vi "Daily_Pass_Fail_Count.vi"(0 "Action":enum16{"READ", "WRITE"}(ring), 5 "Result":bool, 11 "error in":errorcluster) -> (3 "TOTAL":string, 4 "PASS":u32, 6 "FAIL":u32, 8 "PASS":string, 10 "FAIL":string, 15 "error out":errorcluster)   [LabVIEW 2021]
uses:
  controls/INI_Daily_Count_State.ctl
  <vilib>/Utility/config.llb/Write Key (I32).vi
  <vilib>/Utility/config.llb/Write Key (String).vi
  <vilib>/Utility/config.llb/Read Key (String).vi
  <vilib>/Utility/config.llb/Read Key (U32).vi
  <vilib>/Utility/config.llb/Write Key (U32).vi
  <vilib>/Utility/config.llb/NI_LVConfig.lvlib
panel:
  out "appended path":path
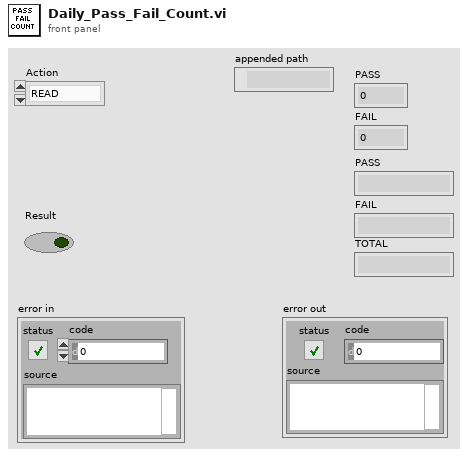
[diagram p1: front panel]
types:
  T1 = typedef "INI_Daily_Count_State.ctl" = enum16{"Check File", "Create INI File", "Check Date", "Read", "Write"}
  T2 = typedef "NI_LVConfig.lvlib/Config Data RefNum.ctl" = refnum<k1>
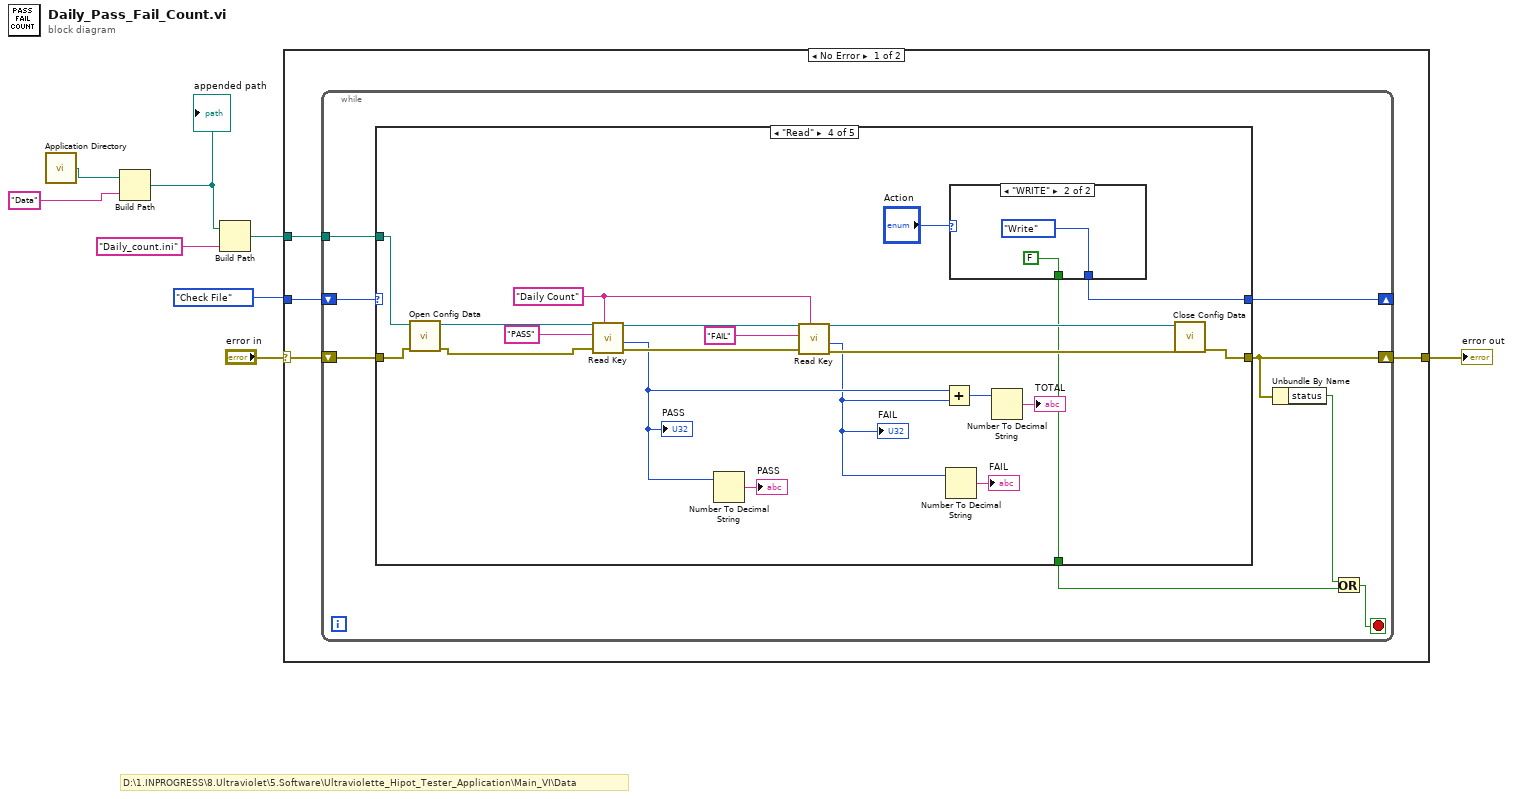
[diagram p0: block diagram]
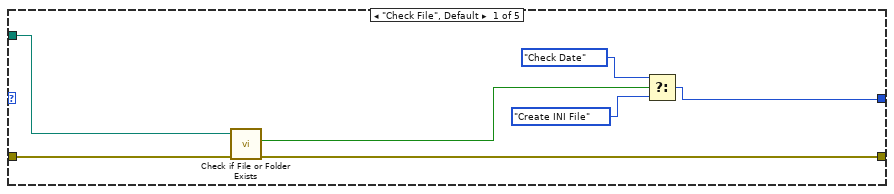
[diagram p2: hidden frame]
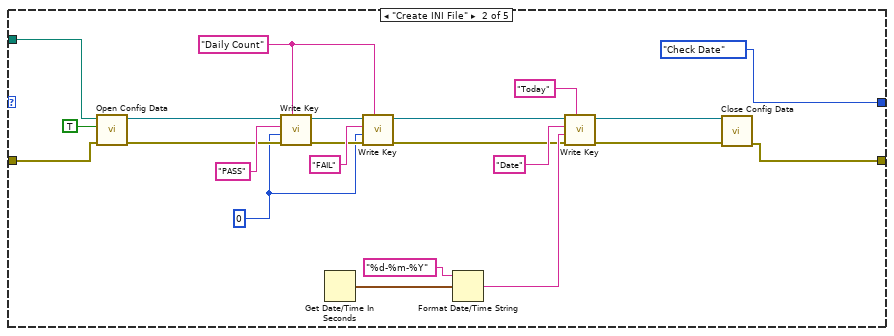
[diagram p3: hidden frame]
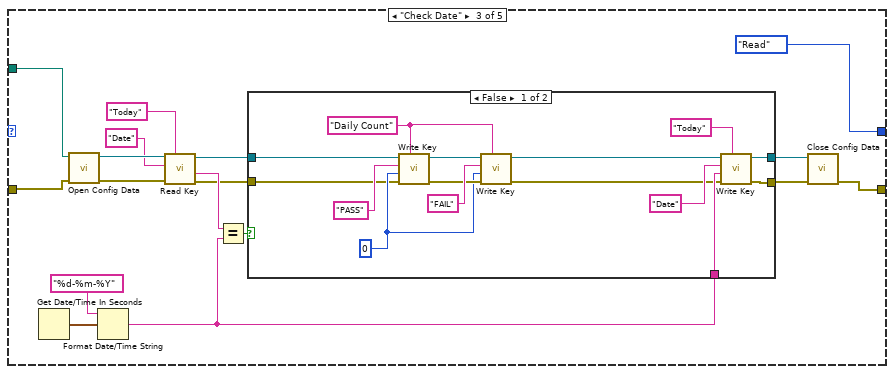
[diagram p4: hidden frame]
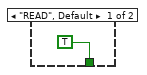
[diagram p6: hidden frame]
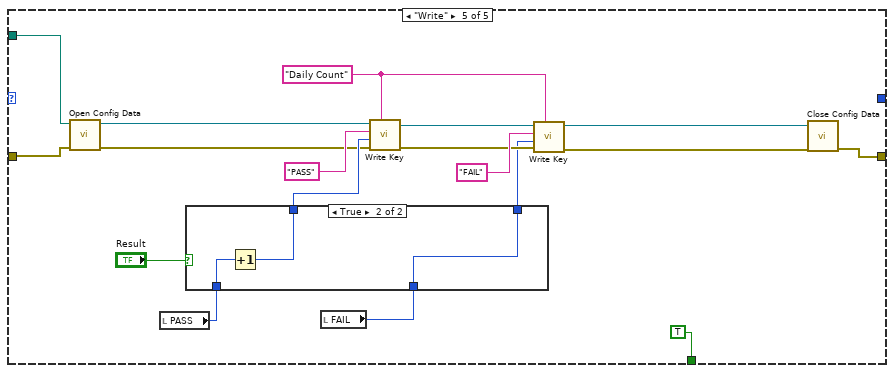
[diagram p7: hidden frame]
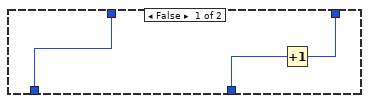
[diagram p8: hidden frame]
diagram:
  # "D:\\1.INPROGRESS\\8.Ultraviolet\\5.Software\\Ultraviolette_Hipot_Tester_Application\\Main_VI\\Data"
  n1 = call <vilib>:"Application Directory.vi"() -> ("Application Directory"=w3:path)
  n2 = Build Path(base path=w3, name or relative path="Data") -> (appended path=w1:path)
  "appended path" <- w1
  n3 = Build Path(base path=w1, name or relative path="Daily_count.ini") -> (appended path=w6:path)
  n4 = case shown="No Error" "error in" {
    selector: "error in" -> [w11 w132]
    tunnel: INI_Daily_Count_State."Check File" -> [w12 _]
    tunnel: [w10 w132] -> w7
    tunnel: w6 -> [w9 _]
    frame No Error {
      n5 = while {
        shift-right: [w19] -> _
        shift-left: w12 -> [w20]
        shift-right: [w15] -> w10
        shift-left: w11 -> [w18]
        tunnel: w9 -> [w17]
        stop <- w16 stop-if-true
        n6 = case shown="\"Read\"" w20 {
          tunnel: [w26 INI_Daily_Count_State."Check Date" INI_Daily_Count_State."Read" w92 _] -> w19
          tunnel: w18 -> [w24 w41 w61 w102 w124]
          tunnel: [w25 w42 w54 w100 w123] -> w15
          tunnel: w17 -> [w23 w40 w62 w103 w125]
          tunnel: [_ _ _ w93 TRUE] -> w13
          frame "Check File", Default {
            n7 = call <vilib>:"Check if File or Folder Exists.vi"("error in (no error)"=w24, "path"=w23) -> ("error out"=w25:errorcluster, "file or folder exists?"=w27:bool)  [unwired: 7 in, 1 out]
            n8 = Select(t=INI_Daily_Count_State."Check Date", s=w27, f=INI_Daily_Count_State."Create INI File") -> (s? t:f=w26:T1)
          }
          frame "Create INI File" {
            w28 = "Daily Count" ("section")
            w37 = 0
            n9 = call <vilib>:"Open Config Data.vi"("error in (no error)"=w41, "create file if necessary (T)"=TRUE, "configuration file path"=w40) -> ("error out"=w46:errorcluster, "refnum"=w48:T2)  [unwired: 6 in, 1 out]
            n10 = call-poly <vilib>:"Write Key.vi"("section"=w28, "error in (no error)"=w46, "value"=w37, "key"="PASS", "refnum"=w48) -> ("error out"=w44:errorcluster, "refnum out"=w43:T2)  [unwired: 4 in, 1 out]
            n11 = Get Date/Time In Seconds() -> (seconds since 1Jan1904=w39:timestamp)
            n12 = call-poly <vilib>:"Write Key.vi"("section"=w28, "error in (no error)"=w44, "value"=w37, "key"="FAIL", "refnum"=w43) -> ("error out"=w29:errorcluster, "refnum out"=w30:T2)  [unwired: 4 in, 1 out]
            n13 = Format Date/Time String(time format string (%c)="%d-%m-%Y", seconds (now)=w39) -> (date/time string=w34:string)  [unwired: 1 in]
            n14 = call-poly <vilib>:"Write Key.vi"("section"="Today", "error in (no error)"=w29, "value"=w34, "key"="Date", "refnum"=w30) -> ("error out"=w32:errorcluster, "refnum out"=w33:T2)  [unwired: 4 in, 1 out]
            n15 = call <vilib>:"Close Config Data.vi"("error in (no error)"=w32, "refnum"=w33) -> ("error out"=w42:errorcluster)  [unwired: 8 in, 1 out]
          }
          frame "Check Date" {
            n16 = Get Date/Time In Seconds() -> (seconds since 1Jan1904=w66:timestamp)
            n17 = call <vilib>:"Open Config Data.vi"("error in (no error)"=w61, "configuration file path"=w62) -> ("error out"=w64:errorcluster, "refnum"=w63:T2)  [unwired: 7 in, 1 out]
            n18 = Format Date/Time String(time format string (%c)="%d-%m-%Y", seconds (now)=w66) -> (date/time string=w56:string)  [unwired: 1 in]
            n19 = call-poly <vilib>:"Read Key.vi"("section"="Today" ("key"), "error in (no error)"=w64, "key"="Date" ("default value"), "refnum"=w63) -> ("error out"=w58:errorcluster, "value"=w60:string, "refnum out"=w57:T2)  [unwired: 4 in, 1 out]
            n20 = Equal?(x=w60, y=w56) -> (x = y?=w59:bool)
            n21 = case shown="False" w59 {
              tunnel: w58 -> [w74 w83]
              tunnel: w57 -> [w73 w82]
              tunnel: [w72 w83] -> w55
              tunnel: w56 -> [w71 _]
              tunnel: [w70 w82] -> w53
              frame False {
                w77 = 0
                w69 = "Daily Count" ("section")
                n22 = call-poly <vilib>:"Write Key.vi"("section"=w69, "error in (no error)"=w74, "value"=w77, "key"="PASS", "refnum"=w73) -> ("error out"=w79:errorcluster, "refnum out"=w78:T2)  [unwired: 4 in, 1 out]
                n23 = call-poly <vilib>:"Write Key.vi"("section"=w69, "error in (no error)"=w79, "value"=w77, "key"="FAIL", "refnum"=w78) -> ("error out"=w67:errorcluster, "refnum out"=w68:T2)  [unwired: 4 in, 1 out]
                n24 = call-poly <vilib>:"Write Key.vi"("section"="Today", "error in (no error)"=w67, "value"=w71, "key"="Date", "refnum"=w68) -> ("error out"=w72:errorcluster, "refnum out"=w70:T2)  [unwired: 4 in, 1 out]
              }
              frame True {
              }
            }
            n25 = call <vilib>:"Close Config Data.vi"("error in (no error)"=w55, "refnum"=w53) -> ("error out"=w54:errorcluster)  [unwired: 8 in, 1 out]
          }
          frame "Read" {
            w90 = "Daily Count" ("section")
            n26 = call <vilib>:"Open Config Data.vi"("error in (no error)"=w102, "configuration file path"=w103) -> ("error out"=w91:errorcluster, "refnum"=w104:T2)  [unwired: 7 in, 1 out]
            n27 = call-poly <vilib>:"Read Key.vi"("section"=w90, "error in (no error)"=w91, "key"="PASS", "refnum"=w104) -> ("error out"=w98:errorcluster, "value"=w87:u32, "refnum out"=w97:T2)  [unwired: 4 in, 1 out]
            "PASS" <- w87
            n28 = Number To Decimal String(number=w87) -> (decimal integer string=→"PASS":string)  [unwired: 1 in]
            n29 = call-poly <vilib>:"Read Key.vi"("section"=w90, "error in (no error)"=w98, "key"="FAIL", "refnum"=w97) -> ("error out"=w96:errorcluster, "value"=w86:u32, "refnum out"=w95:T2)  [unwired: 4 in, 1 out]
            "FAIL" <- w86
            n30 = Add(x=w87, y=w86) -> (x+y=w85:u32)
            n31 = Number To Decimal String(number=w86) -> (decimal integer string=→"FAIL":string)  [unwired: 1 in]
            n32 = case shown="\"WRITE\"" "Action" {
              tunnel: [TRUE FALSE] -> w93
              tunnel: [_ INI_Daily_Count_State."Write"] -> w92
              frame "READ", Default {
              }
              frame "WRITE" {
              }
            }
            n33 = Number To Decimal String(number=w85) -> (decimal integer string=→"TOTAL":string)  [unwired: 1 in]
            n34 = call <vilib>:"Close Config Data.vi"("error in (no error)"=w96, "refnum"=w95) -> ("error out"=w100:errorcluster)  [unwired: 8 in, 1 out]
          }
          frame "Write" {
            w119 = "Daily Count" ("section")
            n35 = call <vilib>:"Open Config Data.vi"("error in (no error)"=w124, "configuration file path"=w125) -> ("error out"=w109:errorcluster, "refnum"=w108:T2)  [unwired: 7 in, 1 out]
            n36 = local read "PASS"() -> (w114:u32)
            n37 = local read "FAIL"() -> (w112:u32)
            n38 = case shown="True" "Result" {
              tunnel: [w128 w131] -> w115
              tunnel: w114 -> [w128 w130]
              tunnel: [w126 w129] -> w113
              tunnel: w112 -> [w127 w129]
              frame False {
                n39 = Increment(x=w127) -> (x+1=w126:u32)
              }
              frame True {
                n40 = Increment(x=w130) -> (x+1=w131:u32)
              }
            }
            n41 = call-poly <vilib>:"Write Key.vi"("section"=w119, "error in (no error)"=w109, "value"=w115, "key"="PASS", "refnum"=w108) -> ("error out"=w117:errorcluster, "refnum out"=w111:T2)  [unwired: 4 in, 1 out]
            n42 = call-poly <vilib>:"Write Key.vi"("section"=w119, "error in (no error)"=w117, "value"=w113, "key"="FAIL", "refnum"=w111) -> ("error out"=w118:errorcluster, "refnum out"=w110:T2)  [unwired: 4 in, 1 out]
            n43 = call <vilib>:"Close Config Data.vi"("error in (no error)"=w118, "refnum"=w110) -> ("error out"=w123:errorcluster)  [unwired: 8 in, 1 out]
          }
        }
        n44 = Unbundle By Name(w15) -> ("status"=w14:bool)
        n45 = Or(x=w14, y=w13) -> (x .or. y?=w16:bool)
      }
    }
    frame Error {
    }
  }
  "error out" <- w7
